vi "step_test.vi"(7 "Stop Button":bool, 8 "轉向":bool, 9 "C/DIO0 (DIO0)":bool, 10 "Period":i64=1000, 11 "error in (no error)":errorcluster) -> ()   [LabVIEW 2019]
uses:
  <vilib>/Platform/TimedLoop/XDataNode/timing_clust.ctl
  <vilib>/Platform/TimedLoop/XDataNode/nitl_modes.ctl
  <vilib>/Platform/TimedLoop/XDataNode/wakeup.ctl
  <vilib>/myRIO/Instrument Drivers/Onboard IO/DIO/typedefs/DIO Reference.ctl
  <vilib>/myRIO/Common/Instrument Driver Framework/Utilities/typedefs/myRIO Generic Hardware Reference.ctl
  <vilib>/myRIO/Common/Instrument Driver Framework/Utilities/typedefs/Hardware Version Enum.ctl
  <vilib>/myRIO/Common/Instrument Driver Framework/Utilities/typedefs/myRIO v1.0 Reference.ctl
  <vilib>/myRIO/Common/Instrument Driver Framework/Utilities/typedefs/Generic FPGA Reference.ctl
  <vilib>/myRIO/Common/Instrument Driver Framework/myRIO v1.0/DIO/typedefs/DIO Channels List.ctl
  <vilib>/myRIO/Common/Instrument Driver Framework/myRIO v1.0/DIO/typedefs/DIO Channels Enum.ctl
  <vilib>/userDefined/High Color/nirio_resource_hc.ctl
  <vilib>/myRIO/Common/Instrument Driver Framework/Utilities/vis/Is FPGA Ref Available.vi
  <vilib>/myRIO/Common/Instrument Driver Framework/myRIO v1.0/DIO/vis/myRIO v1.1 Open DIO.vi
  <vilib>/myRIO/Instrument Drivers/Onboard IO/DIO/vis/Write.vi
  <vilib>/myRIO/Instrument Drivers/Onboard IO/DIO/vis/Read.vi
  <vilib>/myRIO/Common/Instrument Driver Framework/Utilities/vis/Validate Channels.vi
  <vilib>/myRIO/Common/Instrument Driver Framework/myRIO v1.0/DIO/vis/myRIO v1.0 Reserve DIO.vi
  <vilib>/myRIO/Common/Instrument Driver Framework/myRIO v1.0/Resource Manager/vis/myRIO v1.0 Reserve Channel List.vi
  <vilib>/myRIO/Common/Instrument Driver Framework/myRIO v1.0/DIO/vis/myRIO v1.0 Build MUX Configuration DIO.vi
  <vilib>/myRIO/Common/Instrument Driver Framework/myRIO v1.0/Resource Manager/vis/myRIO v1.0 Reserve Channel.vi
  <vilib>/myRIO/Common/Instrument Driver Framework/myRIO v1.0/Resource Manager/vis/myRIO v1.0 Unreserve Channel.vi
  <vilib>/myRIO/Common/Instrument Driver Framework/myRIO v1.0/Resource Manager/vis/myRIO v1.0 Create Configuration List.vi
  <vilib>/myRIO/Common/Instrument Driver Framework/myRIO v1.0/Resource Manager/vis/myRIO v1.0 Build Mutex Name.vi
  <vilib>/Utility/VariantDataType/GetNumericInfo.vi
  <vilib>/Utility/error.llb/Error Cluster From Error Code.vi
  <vilib>/myRIO/Common/Instrument Driver Framework/myRIO v1.0/myRIO v1.1 Open.vi
  <vilib>/myRIO/Common/Instrument Driver Framework/Utilities/vis/IO Manager.vi
  <vilib>/myRIO/Common/Instrument Driver Framework/Utilities/vis/Configuration Manager.vi
  <vilib>/myRIO/Common/Instrument Driver Framework/myRIO v1.0/Resource Manager/vis/myRIO v1.0 Configure IO.vi
  <vilib>/myRIO/Common/Instrument Driver Framework/myRIO v1.0/myRIO v1.0 Close.vi
  <vilib>/myRIO/Common/Instrument Driver Framework/myRIO v1.0/DIO/vis/myRIO v1.0 Write DIO.vi
  <vilib>/myRIO/Common/Instrument Driver Framework/myRIO v1.0/DIO/vis/myRIO v1.0 Read DIO.vi
  <vilib>/platform/TimedLoop/XDataNode/XDataNode.xnode
  <vilib>/myRIO/Express VI/Onboard IO/DO/DO Express VI.xnode
  <vilib>/myRIO/Instrument Drivers/Onboard IO/DIO/vis/myRIO DIO Open.xnode
  <vilib>/myRIO/Express VI/Onboard IO/DI/DI Express VI.xnode
  <vilib>/Platform/TimedLoop/XDataNode/XDNodeRunTimeDep.lvlib
  <vilib>/myRIO/Instrument Drivers/Onboard IO/DIO/DIO.lvlib
panel:
  in  "updown_PWM":bool
  in  "updown":bool
  out "A/DIO6 (Pin 23)":bool
  in  "pushpull_PWM":bool
  in  "pushpull":bool
  out "B/DIO5 (Pin 21)":bool
  in  "4":bool
  in  "3":bool
  in  "同向":bool
  out "s? t:f":dbl
  out "Numeric":i32
  # "true上"
  # "T推\nF拉"
  # "T上\nF下"
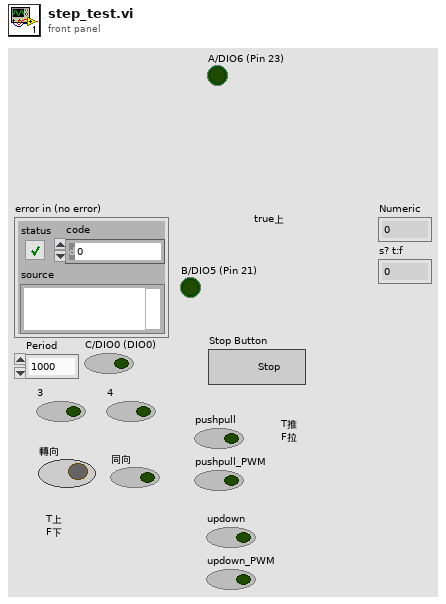
[diagram p1: front panel]
types:
  T1 = typedef "XDNodeRunTimeDep.lvlib/timing_clust.ctl" = cluster{"Expected End [f-1]":u64, "Actual End [f-1]":u64, "Finished Late? [f-1]":bool, "Expected End [i-1]":u64, "Actual End [i-1]":u64, "Finished Late? [i-1]":bool, "Expected Start [i]":u64, "Actual Start [i]":u64, "Expected Start [f]":u64, "Actual Start [f]":u64, "Source Name":string, "Structure Name":string, "Period":i64, "Deadline":i64, "Offset":i64, "Start":i64, "Priority":i32, "Timeout":i32, "Mode":T2, "Wakeup Reason":T3, "Error":errorcluster, "Source Type":string, "Secondary Source Type":string, "Global End Time":u64, "Global Start Time":u64, "Frame Duration":u64, "Iteration Duration":u64, "Assigned CPU":i32, "I/O Scan Engine Mode":u32}
  T2 = typedef "XDNodeRunTimeDep.lvlib/nitl_modes.ctl" = enum32{"No Change", "Process missed periods, maintain original phase", "Discard missed periods, maintain original phase", "Process missed periods, ignore original phase", "Discard missed periods, ignore original phase"}
  T3 = typedef "XDNodeRunTimeDep.lvlib/wakeup.ctl" = enum32{"Normal", "Aborted", "Asynchronous wakeup", "Timing source error", "Timed loop error", "Timeout"}
  T4 = typedef "DIO.lvlib/DIO Reference.ctl" = cluster{"myRIO Reference":T5, "DIO Channels List":T9}
  T5 = typedef "myRIO Generic Hardware Reference.ctl" = cluster{"myRIO Model":T6, "myRIO Hardware Reference":T7}
  T6 = typedef "Hardware Version Enum.ctl" = enum16{"Unknown", "myRIO-1900", "myRIO-1950", "roboRIO", "NI ELVIS RIO CM", "ELVIS III"}
  T7 = typedef "myRIO v1.0 Reference.ctl" = cluster{"Generic FPGA Reference":T8, "Allow multiple opens":bool}
  T8 = typedef "Generic FPGA Reference.ctl" = refnum<k20>
  T9 = typedef "DIO Channels List.ctl" = T10[]
  T10 = typedef "DIO Channels Enum.ctl" = enum16{"Not Connected", "C/DIO0", "C/DIO1", "C/DIO2", "C/DIO3", "C/DIO4", "C/DIO5", "C/DIO6", "C/DIO7", "A/DIO0", "A/DIO1", "A/DIO2", "A/DIO3", "A/DIO4", "A/DIO5", "A/DIO6", "A/DIO7", "A/DIO8", "A/DIO9", "A/DIO10", "A/DIO11", "A/DIO12", "A/DIO13", "A/DIO14", "A/DIO15", "A/DIO16", "A/DIO17", "A/DIO18", "A/DIO19", "B/DIO0", "B/DIO1", "B/DIO2", "B/DIO3", "B/DIO4", "B/DIO5", "B/DIO6", "B/DIO7", "B/DIO8", "B/DIO9", "B/DIO10", "B/DIO11", "B/DIO12", "B/DIO13", "B/DIO14", "B/DIO15", "B/DIO16", "B/DIO17", "B/DIO18", "B/DIO19", "LED0", "LED1", "LED2", "LED3", "Button0", "DIO/DIO0", "DIO/DIO1", "DIO/DIO2", "DIO/DIO3", "DIO/DIO4", "DIO/DIO5", "DIO/DIO6", "DIO/DIO7", "DIO/DIO8", "DIO/DIO9", "SPI/CS0", "SPI/CS1", "SPI/CS2", "SPI/CS3", "LED RADIO (Green)", "LED RADIO (Red)", "LED COMM (Green)", "LED COMM (Red)", "LED MODE (Green)", "LED MODE (Red)"}
  T11 = typedef "nirio_resource_hc.ctl" = tag
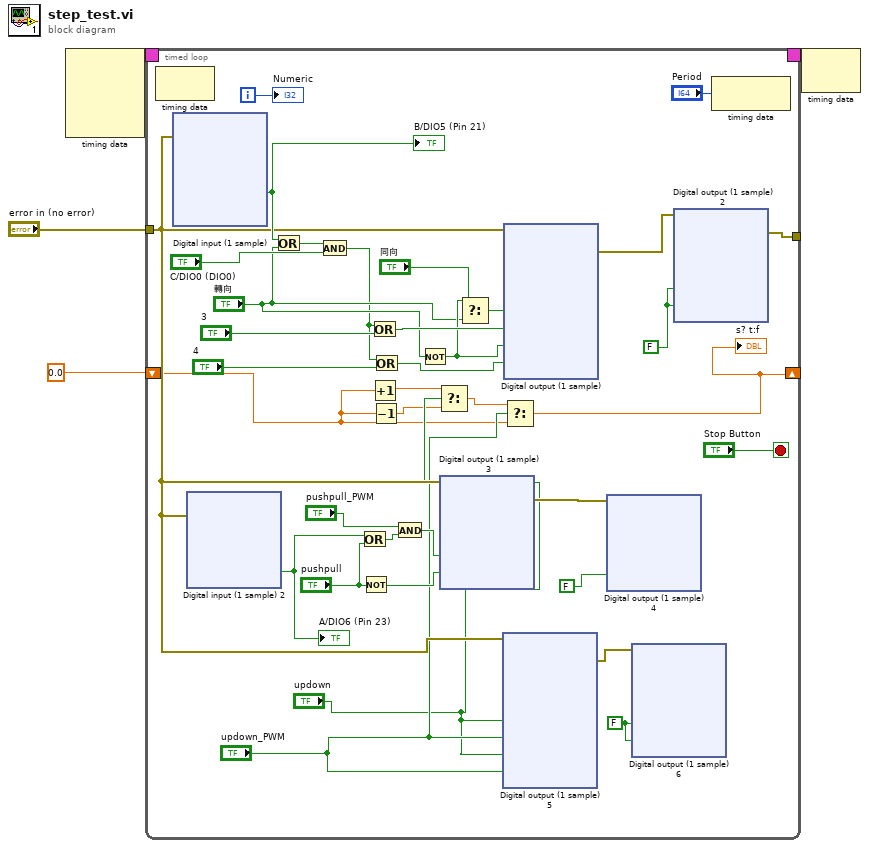
[diagram p0: block diagram]
diagram:
  n1 = node-c288() -> (w4:T1)  [unwired: 4 in]
  n2 = timed-loop {
    timing: w4 -> [_]
    timing-out: [_] -> w3
    tunnel: "error in (no error)" -> [w16]
    shift-right: [w5] -> _
    shift-left: 0.0 -> [w7]
    tunnel: [w36] -> _
    i -> [w38]
    stop <- "Stop Button" stop-if-true
    w15 = FALSE ("RUD_PWM (A/DIO14 (Pin 32))")
    w35 = FALSE ("C/DIO0 (DIO0)")
    n3 = node-c288() -> ()  [unwired: 1 in, 1 out]
    n4 = xnode "Digital input (1 sample)"("error in (no error)"=w16) -> ("B/DIO5 (Pin 21)"=w26:bool)  [unwired: 2 out]
    "B/DIO5 (Pin 21)" <- w26
    n5 = xnode "Digital input (1 sample) 2"("error in (no error)"=w16) -> ("A/DIO6 (Pin 23)"=w19:bool)  [unwired: 1 out]
    "A/DIO6 (Pin 23)" <- w19
    n6 = Or(x=w26, y="轉向") -> (x .or. y?=w27:bool)
    n7 = And(x=w27, y="C/DIO0 (DIO0)") -> (x .and. y?=w18:bool)
    n8 = Or(x=w19, y="pushpull") -> (x .or. y?=w20:bool)
    n9 = Not(x="pushpull") -> (.not. x?=w13:bool)
    n10 = Or(x=w18, y="3") -> (x .or. y?=w30:bool)
    n11 = Increment(x=w7) -> (x+1=w8:dbl)
    n12 = Decrement(x=w7) -> (x-1=w9:dbl)
    n13 = Or(x=w18, y="4") -> (x .or. y?=w29:bool)
    n14 = And(x="pushpull_PWM", y=w20) -> (x .and. y?=w14:bool)
    n15 = Not(x="轉向") -> (.not. x?=w25:bool)
    n16 = Select(t=w8, s="updown", f=w9) -> (s? t:f=w6:dbl)
    n17 = xnode "Digital output (1 sample) 3"("pushpull_PWM (B/DIO6 (Pin 23))"=w14, "pushpull (C/DIO7 (DIO7))"=w13, "error in (no error)"=w16) -> ("error out"=w28:errorcluster)
    n18 = Select(t=w25, s="同向", f="轉向") -> (s? t:f=w23:bool)
    n19 = xnode "Digital output (1 sample) 5"("RUD (A/DIO15 (Pin 34))"="updown", "RUD_PWM (A/DIO14 (Pin 32))"="updown_PWM", "LUD (C/DIO1 (DIO1))"="updown", "LUD_PWM (C/DIO5 (DIO5))"="updown_PWM", "error in (no error)"=w16) -> ("error out"=w17:errorcluster)
    n20 = xnode "Digital output (1 sample)"("3 (B/DIO8 (Pin 27))"=w23, "3_PWM (C/DIO0 (DIO0))"=w30, "4 (B/DIO9 (Pin 29))"=w25, "4_PWM (C/DIO4 (DIO4))"=w29, "error in (no error)"=w16) -> ("error out"=w37:errorcluster)
    n21 = Select(t=w6, s="updown_PWM", f=w7) -> (s? t:f=w5:dbl)
    "s? t:f" <- w5
    n22 = xnode "Digital output (1 sample) 4"("pushpull_PWM (B/DIO6 (Pin 23))"=FALSE ("pushpull (B/DIO6 (Pin 23))"), "error in (no error)"=w28) -> ()  [unwired: 1 out]
    n23 = xnode "Digital output (1 sample) 6"("RUD_PWM (A/DIO14 (Pin 32))"=w15, "LUD_PWM (C/DIO5 (DIO5))"=w15, "error in (no error)"=w17) -> ()  [unwired: 1 out]
    n24 = xnode "Digital output (1 sample) 2"("3 (C/DIO0 (DIO0))"=w35, "4 (C/DIO4 (DIO4))"=w35, "error in (no error)"=w37) -> ("error out"=w36:errorcluster)
    n25 = node-c288("Period") -> ()  [unwired: 1 out]
    "Numeric" <- w38
  }
  n26 = node-c288(w3) -> ()  [unwired: 1 out]
